vi "Lire regulateur MODBUS EPC3000.vi"(3 "error in (no error)":errorcluster caption="entrée d'erreur (pas d'erreur)", 4 "Adresse régulateur":u8=1 min=1 max=16 step=1, 5 "Port COM run 1 REG":refnum<visa-resource-name>) -> (0 "error out":errorcluster caption="entrée d'erreur (pas d'erreur)", 2 "Config + Programmes":T1 {"Programmation configuration"."?" format="%.2f"})   [LabVIEW 2022 SP3]
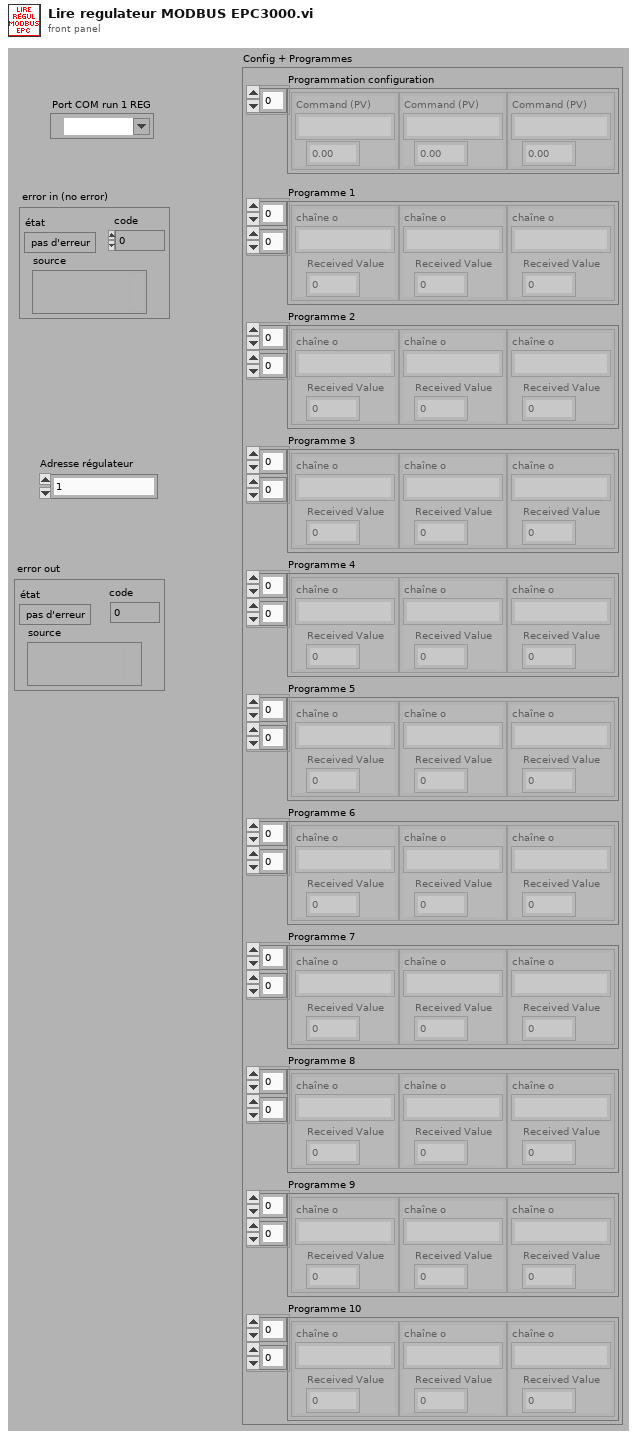
[diagram p1: front panel]
types:
  T1 = cluster{"Programmation configuration":cluster{"Command (PV)":string, dbl}[], "Programme 1":cluster{"chaîne o":string, "Received Value":dbl}[][], "Programme 2":cluster{"chaîne o":string, "Received Value":dbl}[][], "Programme 3":cluster{"chaîne o":string, "Received Value":dbl}[][], "Programme 4":cluster{"chaîne o":string, "Received Value":dbl}[][], "Programme 5":cluster{"chaîne o":string, "Received Value":dbl}[][], "Programme 6":cluster{"chaîne o":string, "Received Value":dbl}[][], "Programme 7":cluster{"chaîne o":string, "Received Value":dbl}[][], "Programme 8":cluster{"chaîne o":string, "Received Value":dbl}[][], "Programme 9":cluster{"chaîne o":string, "Received Value":dbl}[][], "Programme 10":cluster{"chaîne o":string, "Received Value":dbl}[][]}
  T2 = cluster{"chaîne o":string, "Received Value":dbl}[][]
  T3 = cluster{"Programmation configuration":cluster{"Command (PV)":string, dbl}[], "Programme":cluster{"chaîne o":string, "Received Value":dbl}[][], "Programme":cluster{"chaîne o":string, "Received Value":dbl}[][], "Programme":cluster{"chaîne o":string, "Received Value":dbl}[][], "Programme":cluster{"chaîne o":string, "Received Value":dbl}[][], "Programme":cluster{"chaîne o":string, "Received Value":dbl}[][], "Programme":cluster{"chaîne o":string, "Received Value":dbl}[][], "Programme":cluster{"chaîne o":string, "Received Value":dbl}[][], "Programme":cluster{"chaîne o":string, "Received Value":dbl}[][], "Programme":cluster{"chaîne o":string, "Received Value":dbl}[][], "Programme":cluster{"chaîne o":string, "Received Value":dbl}[][]}
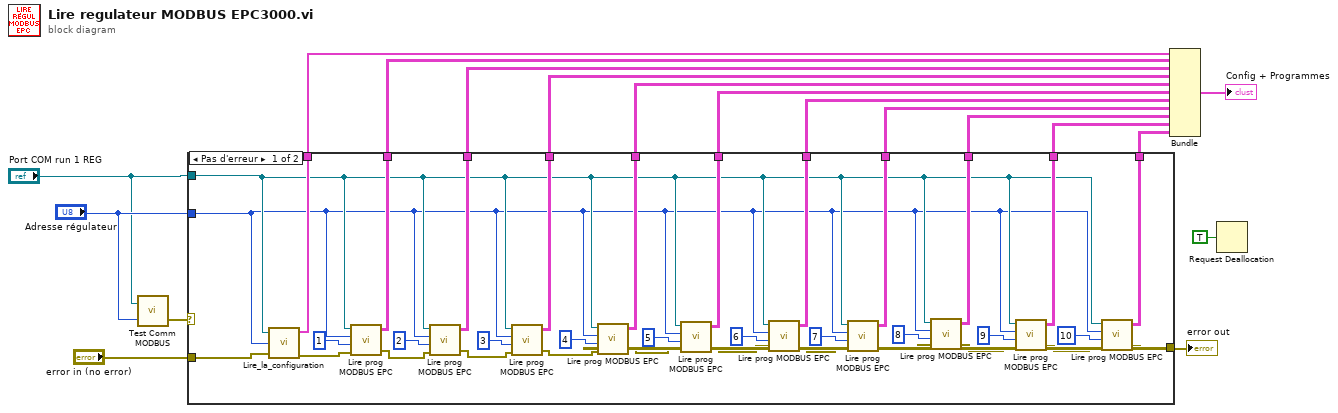
[diagram p0: block diagram]
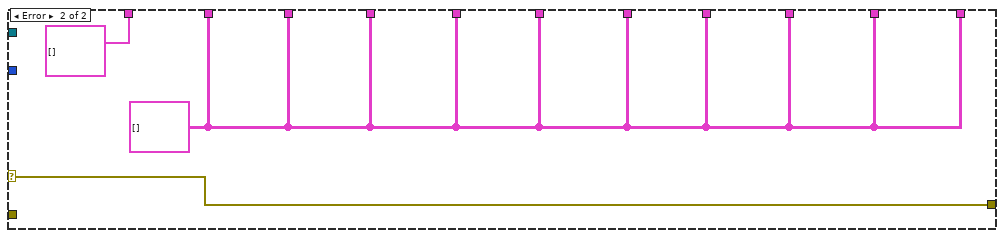
[diagram p2: hidden frame]
diagram:
  n1 = call "Test Comm MODBUS.vi"("Adresse rég"="Adresse régulateur", "Port COM run 1 REG"="Port COM run 1 REG") -> ("error out"=w15:errorcluster)  [unwired: 1 in]
  n2 = case shown="Pas d'erreur" w15 {
    selector: w15 -> [_ w55]
    tunnel: "Adresse régulateur" -> [w26 _]
    tunnel: [w53 cluster{"Command (PV)":string, dbl}[] [] ("Programmation configuration")] -> w12
    tunnel: [w52 w54] -> w11
    tunnel: [w51 w54] -> w10
    tunnel: [w50 w54] -> w9
    tunnel: [w49 w54] -> w8
    tunnel: "error in (no error)" -> [w48 _]
    tunnel: [w19 w55] -> w13
    tunnel: "Port COM run 1 REG" -> [w27 _]
    tunnel: [w38 w54] -> w6
    tunnel: [w37 w54] -> w5
    tunnel: [w34 w54] -> w4
    tunnel: [w33 w54] -> w3
    tunnel: [w30 w54] -> w2
    tunnel: [w29 w54] -> w1
    frame No Error {
      n3 = call "Lire_la_configuration.vi"("Port COM run 1 REG"=w27, "Adresse rég"=w26, "error in (no error)"=w48) -> ("Programmation configuration"=w53:cluster{"Command (PV)":string, dbl}[], "error out"=w45:errorcluster)  [unwired: 2 out]
      n4 = call "Lire prog MODBUS EPC.vi"("error in (no error)"=w45, "Numéro de programme"=u8 1, "Adresse rég"=w26, "Port COM run 1 REG"=w27) -> ("error out"=w47:errorcluster, "Programme"=w52:T2)  [unwired: 1 out]
      n5 = call "Lire prog MODBUS EPC.vi"("error in (no error)"=w47, "Numéro de programme"=u8 2, "Adresse rég"=w26, "Port COM run 1 REG"=w27) -> ("error out"=w44:errorcluster, "Programme"=w51:T2)  [unwired: 1 out]
      n6 = call "Lire prog MODBUS EPC.vi"("error in (no error)"=w44, "Numéro de programme"=u8 3, "Adresse rég"=w26, "Port COM run 1 REG"=w27) -> ("error out"=w43:errorcluster, "Programme"=w50:T2)  [unwired: 1 out]
      n7 = call "Lire prog MODBUS EPC.vi"("error in (no error)"=w43, "Numéro de programme"=u8 4, "Adresse rég"=w26, "Port COM run 1 REG"=w27) -> ("error out"=w25:errorcluster, "Programme"=w49:T2)  [unwired: 1 out]
      n8 = call "Lire prog MODBUS EPC.vi"("error in (no error)"=w25, "Numéro de programme"=u8 5, "Adresse rég"=w26, "Port COM run 1 REG"=w27) -> ("error out"=w24:errorcluster, "Programme"=w38:T2)  [unwired: 1 out]
      n9 = call "Lire prog MODBUS EPC.vi"("error in (no error)"=w24, "Numéro de programme"=u8 6, "Adresse rég"=w26, "Port COM run 1 REG"=w27) -> ("error out"=w23:errorcluster, "Programme"=w37:T2)  [unwired: 1 out]
      n10 = call "Lire prog MODBUS EPC.vi"("error in (no error)"=w23, "Numéro de programme"=u8 7, "Adresse rég"=w26, "Port COM run 1 REG"=w27) -> ("error out"=w22:errorcluster, "Programme"=w34:T2)  [unwired: 1 out]
      n11 = call "Lire prog MODBUS EPC.vi"("error in (no error)"=w22, "Numéro de programme"=u8 8, "Adresse rég"=w26, "Port COM run 1 REG"=w27) -> ("error out"=w21:errorcluster, "Programme"=w33:T2)  [unwired: 1 out]
      n12 = call "Lire prog MODBUS EPC.vi"("error in (no error)"=w21, "Numéro de programme"=u8 9, "Adresse rég"=w26, "Port COM run 1 REG"=w27) -> ("error out"=w20:errorcluster, "Programme"=w30:T2)  [unwired: 1 out]
      n13 = call "Lire prog MODBUS EPC.vi"("error in (no error)"=w20, "Numéro de programme"=u8 10, "Adresse rég"=w26, "Port COM run 1 REG"=w27) -> ("error out"=w19:errorcluster, "Programme"=w29:T2)  [unwired: 1 out]
    }
    frame Error {
      w54 = T2 [] ("Programme")
    }
  }
  "error out" <- w13
  n14 = Bundle("Programmation configuration"=w12, "Programme"=w11, "Programme"=w10, "Programme"=w9, "Programme"=w8, "Programme"=w6, "Programme"=w5, "Programme"=w4, "Programme"=w3, "Programme"=w2, "Programme"=w1) -> (→"Config + Programmes":T3)  [unwired: 1 in]
  n15 = Request Deallocation(TRUE ("flag")) -> ()
